vi "Scan Engine EtherCAT Generic Slave.vi"(8 "error in (no error)":errorcluster, 11 "Node Ptr":T1 format="%.0x") -> (0 "error out":errorcluster)   [LabVIEW 2027, in "SEECD System Explorer.lvlib"]
uses:
  SEECD System Explorer.lvlib
  <vilib>/NI VeriStand/Custom Device API/Custom Device Item Ref.ctl
  Shared/Globals/Property Strings.vi
  <vilib>/NI VeriStand/Custom Device API/Set Item Property (U16).vi
  <vilib>/NI VeriStand/Custom Device API/Set Item Property (Boolean).vi
  <vilib>/NI VeriStand/Custom Device API/Custom Device API.lvlib
  Shared/SEECD Shared.lvlib
  C:/NetCoreDLL/NationalInstruments.VeriStand.SystemDefinitionAPI.dll
  NetCoreDLL/NationalInstruments.VeriStand.SystemDefinitionAPI.dll
panel:
  in  "Enable Distributed Clock":bool caption="Enable distributed clock"
  out "ToString":string
  in  "Export to XML":bool
  in  "Prepend":bool caption="Prepend slave position to name"
  in  "SHDocVw.IWebBrowser2":refnum<k7>(container)
  in  "Slave Position":u16
  in  "Header":cluster{"Section Name":string}={"Section Name"="EtherCAT Slave"}
  in  "Name":string
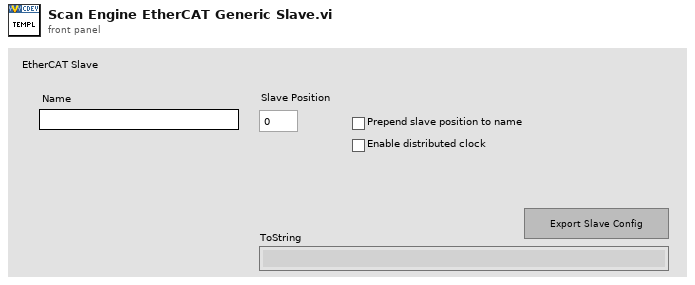
[diagram p1: front panel]
types:
  T1 = typedef "Custom Device API.lvlib/Custom Device Item Ref.ctl" = u64
  T2 = typedef "Custom Device API.lvlib/Custom Device Commands.ctl" = enum16{"Default", "Item renamed", "Shutdown", "Dynamic button pressed"}
  T3 = typedef "Custom Device API.lvlib/Custom Device Pointer.ctl" = refnum<k39>
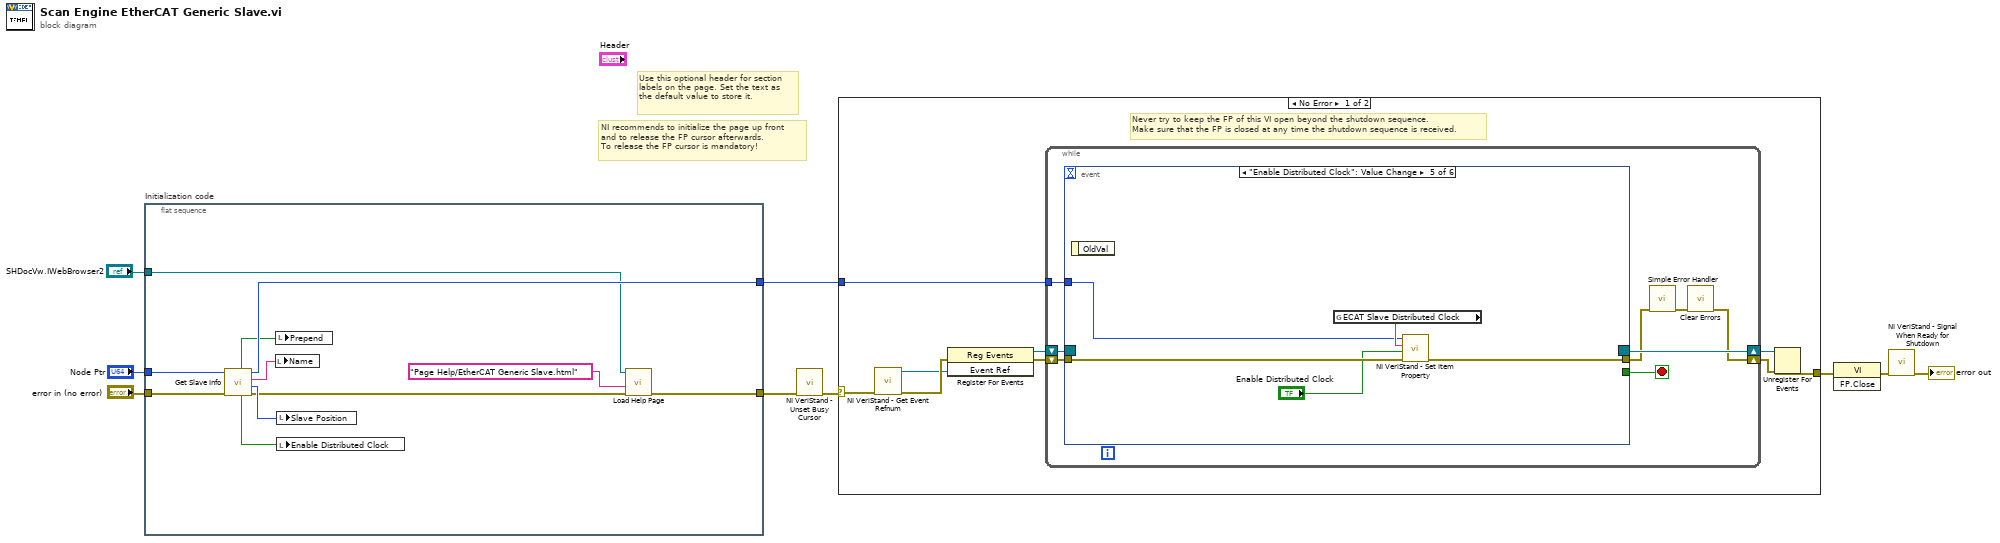
[diagram p0: block diagram]
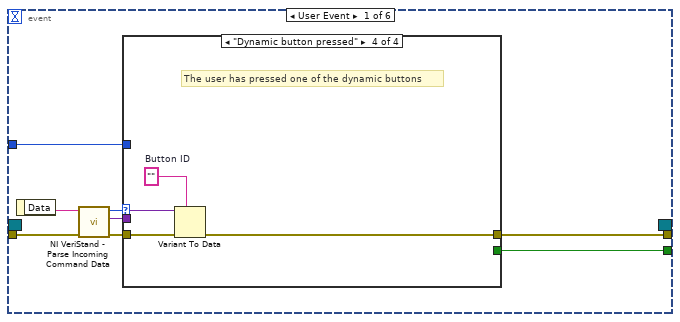
[diagram p2: hidden frame]
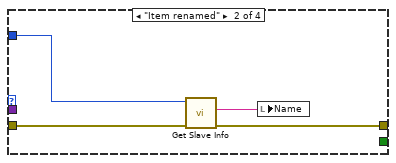
[diagram p4: hidden frame]
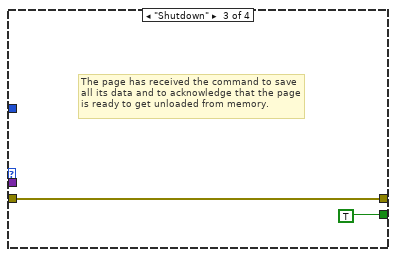
[diagram p5: hidden frame]
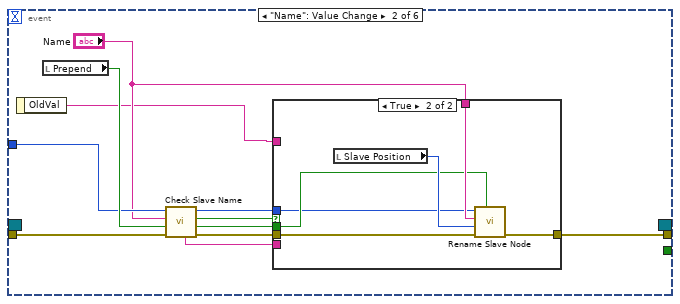
[diagram p6: hidden frame]
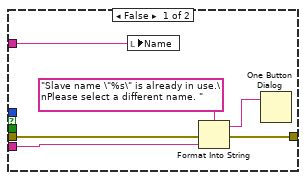
[diagram p7: hidden frame]
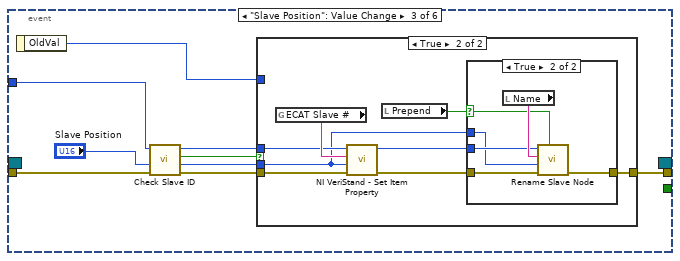
[diagram p8: hidden frame]
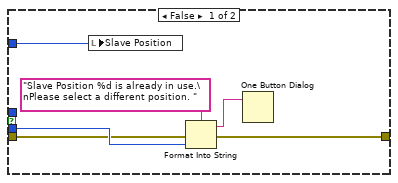
[diagram p9: hidden frame]
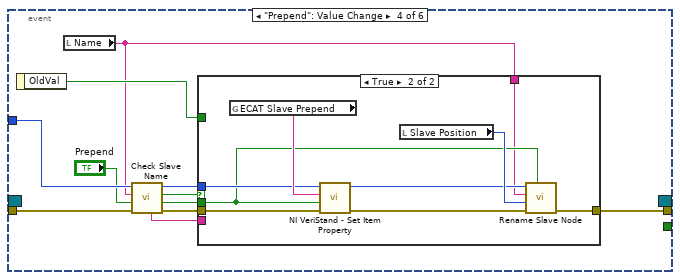
[diagram p11: hidden frame]
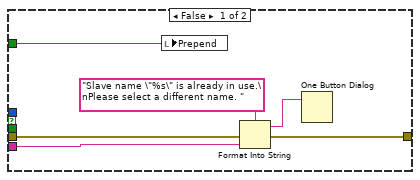
[diagram p12: hidden frame]
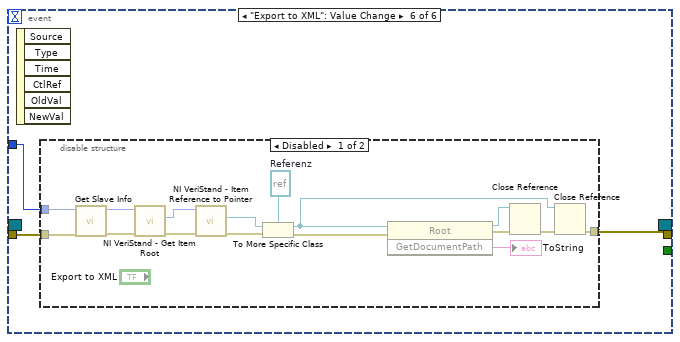
[diagram p13: hidden frame]
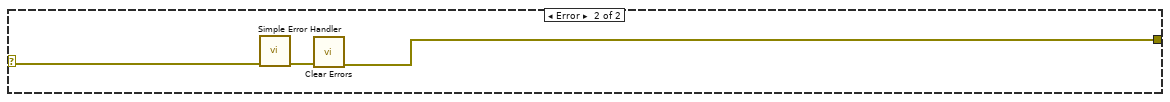
[diagram p15: hidden frame]
diagram:
  # "Use this optional header for section labels on the page. Set the text as the default value to store it."
  # "NI recommends to initialize the page up front\nand to release the FP cursor afterwards.\nTo release the FP cursor is mandatory!"
  n1 = flat-sequence "Initialization code" {
    tunnel: "error in (no error)" -> [w16]
    tunnel: "Node Ptr" -> [w17]
    tunnel: [w18] -> w3
    tunnel: "SHDocVw.IWebBrowser2" -> [w11]
    tunnel: [w12] -> w1
    frame #0 {
      n2 = call "Get Slave Info.vi"("error in (no error)"=w16, "Item Ref in"=w17) -> ("error out"=w13:errorcluster, "Slave #"=w19:u16, "Slave Name"=w20:string, "Item Ref out"=w18:T1, "Distributed Clock"=w10:bool, "Prepend"=w15:bool)  [unwired: 4 in]
      n3 = local write "Name"(w20) -> ()
      n4 = local write "Prepend"(w15) -> ()
      n5 = local write "Slave Position"(w19) -> ()
      n6 = local write "Enable Distributed Clock"(w10) -> ()
      n7 = call "Load Help Page.vi"("error in (no error)"=w13, "HTML File to Load"="Page Help/EtherCAT Generic Slave.html" ("name or relative path"), "Browser"=w11) -> ("error out"=w12:errorcluster)  [unwired: 8 in]
    }
  }
  n8 = call <vilib>:"NI VeriStand - Unset Busy Cursor.vi"("error in (no error)"=w1) -> ("error out"=w5:errorcluster)  [unwired: 10 out]
  n9 = case shown="No Error" w5 {
    selector: w5 -> [w21 w162]
    tunnel: [w26 w160] -> w9
    tunnel: w3 -> [w22 _]
    frame No Error {
      # "Never try to keep the FP of this VI open beyond the shutdown sequence.\nMake sure that the FP is closed at any time the shutdown sequence is received."
      n10 = call <vilib>:"NI VeriStand - Get Event Refnum.vi"("error in (no error)"=w21) -> ("error out"=w29:errorcluster, "Event Ref"=w25:refnum<user-event>)  [unwired: 9 out]
      n11 = register-events(error in=w29, w25) -> (reference out=w23:refnum<event-registration>, error out=w24:errorcluster)  [unwired: 1 in]
      n12 = while {
        tunnel: w22 -> [w33]
        shift-right: [w30] -> w27
        shift-left: w24 -> [w36]
        shift-right: [w37] -> w28
        shift-left: w23 -> [w35]
        stop <- w34 stop-if-true
        n13 = event shown="[4] \"Enable Distributed Clock\": Value Change" {
          selector: w35 -> [_ _ _ _ _ _]
          dyn-events: [_ _ _ _ _ _] -> w37
          timeout: _ -> [_ _ _ _ _ _]
          tunnel: w36 -> [w45 w60 w82 w118 w139 w143]
          tunnel: [w41 _ _ _ _ _] -> w34
          tunnel: [w40 w59 w80 w119 w138 w141] -> w32
          tunnel: w33 -> [w39 w61 w84 w117 w137 w142]
          event User Event {
            n14 = event-data() -> ("Data"=w44:string)  [unwired: 1 out]
            n15 = call <vilib>:"NI VeriStand - Parse Incoming Command Data.vi"("error in (no error)"=w45, "Incoming data"=w44) -> ("error out"=w43:errorcluster, "Outgoing data"=w38:variant, "Action"=w42:T2)  [unwired: 7 out]
            n16 = case shown="\"Dynamic button pressed\"" w42 {
              tunnel: w43 -> [w46 w50 w51 w56]
              tunnel: [_ _ TRUE _] -> w41
              tunnel: [w46 w49 w51 w53] -> w40
              tunnel: w39 -> [_ w47 _ _]
              tunnel: w38 -> [_ _ _ w55]
              frame "Default", Default {
              }
              frame "Item renamed" {
                n17 = call "Get Slave Info.vi"("error in (no error)"=w50, "Item Ref in"=w47) -> ("error out"=w49:errorcluster, "Slave Name"=w48:string)  [unwired: 4 in, 4 out]
                n18 = local write "Name"(w48) -> ()
              }
              frame "Shutdown" {
                # "The page has received the command to save all its data and to acknowledge that the page is ready to get unloaded from memory."
              }
              frame "Dynamic button pressed" {
                w54 = ""  # Button ID
                # "The user has pressed one of the dynamic buttons"
                n19 = Variant To Data(error in=w56, type=w54, Variant=w55) -> (error out=w53:errorcluster)  [unwired: 1 out]
              }
            }
          }
          event "Name": Value Change {
            n20 = event-data() -> ("OldVal"=w57:string)  [unwired: 1 out]
            n21 = local read "Prepend"() -> (w62:bool)
            n22 = call "Check Slave Name.vi"("error in (no error)"=w60, "Prepend in"=w62, "Slave Name In"="Name", "Item Ref in"=w61) -> ("error out"=w65:errorcluster, "Prepend out"=w64:bool, "Available?"=w66:bool, "Item Ref out"=w67:T1, "Slave Name"=w63:string)  [unwired: 3 in]
            n23 = case shown="True" w66 {
              tunnel: [w71 w79] -> w59
              tunnel: w65 -> [w72 w76]
              tunnel: w67 -> [_ w74]
              tunnel: w64 -> [_ w75]
              tunnel: w63 -> [w69 _]
              tunnel: "Name" -> [_ w77]
              tunnel: w57 -> [w68 _]
              frame False {
                n24 = local write "Name"(w68) -> ()
                n25 = Format Into String(format string="Slave name \"%s\" is already in use.\nPlease select a different name. ", error in=w72, w69) -> (resulting string=w70:string, error out=w71:errorcluster)  [unwired: 1 in]
                n26 = One Button Dialog(message=w70) -> ()  [unwired: 1 in, 1 out]
              }
              frame True {
                n27 = local read "Slave Position"() -> (w78:u16)
                n28 = call "Rename Slave Node.vi"("Prepend"=w75, "error in (no error)"=w76, "Slave #"=w78, "Slave Name"=w77, "Item Ref in"=w74) -> ("error out"=w79:errorcluster)  [unwired: 5 in, 1 out]
              }
            }
          }
          event "Slave Position": Value Change {
            n29 = event-data() -> ("OldVal"=w81:u16)  [unwired: 1 out]
            n30 = call "Check Slave ID.vi"("error in (no error)"=w82, "Slave ID in"="Slave Position", "Item Ref in"=w84) -> ("error out"=w88:errorcluster, "Slave ID out"=w86:u16, "Available?"=w87:bool, "Item Ref out"=w85:T1)  [unwired: 5 in]
            n31 = case shown="True" w87 {
              tunnel: [w90 w102] -> w80
              tunnel: w88 -> [w91 w100]
              tunnel: w85 -> [_ w98]
              tunnel: w86 -> [w93 w96]
              tunnel: w81 -> [w89 _]
              frame False {
                n32 = local write "Slave Position"(w89) -> ()
                n33 = Format Into String(format string="Slave Position %d is already in use.\nPlease select a different position. ", error in=w91, w93) -> (resulting string=w92:string, error out=w90:errorcluster)  [unwired: 1 in]
                n34 = One Button Dialog(message=w92) -> ()  [unwired: 1 in, 1 out]
              }
              frame True {
                n35 = global read "Property Strings.vi" "ECAT Slave #"() -> (w101:string)
                n36 = call-poly <vilib>:"NI VeriStand - Set Item Property.vi"("error in (no error)"=w100, "Value"=w96, "Property Name"=w101, "Item Ref in"=w98) -> ("error out"=w99:errorcluster, "Item Ref out"=w97:T1)  [unwired: 5 in, 1 out]
                n37 = local read "Prepend"() -> (w95:bool)
                n38 = case shown="True" w95 {
                  selector: w95 -> [_ w104]
                  tunnel: [w103 w109] -> w102
                  tunnel: w99 -> [w103 w107]
                  tunnel: w97 -> [_ w106]
                  tunnel: w96 -> [_ w105]
                  frame False {
                  }
                  frame True {
                    n39 = local read "Name"() -> (w108:string)
                    n40 = call "Rename Slave Node.vi"("Prepend"=w104, "error in (no error)"=w107, "Slave #"=w105, "Slave Name"=w108, "Item Ref in"=w106) -> ("error out"=w109:errorcluster)  [unwired: 5 in, 1 out]
                  }
                }
              }
            }
          }
          event "Prepend": Value Change {
            n41 = event-data() -> ("OldVal"=w120:bool)  [unwired: 1 out]
            n42 = local read "Name"() -> (w110:string)
            n43 = call "Check Slave Name.vi"("error in (no error)"=w118, "Prepend in"="Prepend", "Slave Name In"=w110, "Item Ref in"=w117) -> ("error out"=w113:errorcluster, "Prepend out"=w112:bool, "Available?"=w114:bool, "Item Ref out"=w115:T1, "Slave Name"=w111:string)  [unwired: 3 in]
            n44 = case shown="True" w114 {
              tunnel: [w123 w135] -> w119
              tunnel: w113 -> [w124 w132]
              tunnel: w115 -> [_ w130]
              tunnel: w112 -> [_ w128]
              tunnel: w120 -> [w126 _]
              tunnel: w111 -> [w121 _]
              tunnel: w110 -> [_ w127]
              frame False {
                n45 = local write "Prepend"(w126) -> ()
                n46 = Format Into String(format string="Slave name \"%s\" is already in use.\nPlease select a different name. ", error in=w124, w121) -> (resulting string=w122:string, error out=w123:errorcluster)  [unwired: 1 in]
                n47 = One Button Dialog(message=w122) -> ()  [unwired: 1 in, 1 out]
              }
              frame True {
                n48 = global read "Property Strings.vi" "ECAT Slave Prepend"() -> (w133:string)
                n49 = call-poly <vilib>:"NI VeriStand - Set Item Property.vi"("error in (no error)"=w132, "Value"=w128, "Property Name"=w133, "Item Ref in"=w130) -> ("error out"=w131:errorcluster, "Item Ref out"=w129:T1)  [unwired: 5 in, 1 out]
                n50 = local read "Slave Position"() -> (w134:u16)
                n51 = call "Rename Slave Node.vi"("Prepend"=w128, "error in (no error)"=w131, "Slave #"=w134, "Slave Name"=w127, "Item Ref in"=w129) -> ("error out"=w135:errorcluster)  [unwired: 5 in, 1 out]
              }
            }
          }
          event "Enable Distributed Clock": Value Change {
            n52 = event-data() -> ()  [unwired: 2 out]
            n53 = global read "Property Strings.vi" "ECAT Slave Distributed Clock"() -> (w140:string)
            n54 = call-poly <vilib>:"NI VeriStand - Set Item Property.vi"("error in (no error)"=w139, "Value"="Enable Distributed Clock", "Property Name"=w140, "Item Ref in"=w137) -> ("error out"=w138:errorcluster)  [unwired: 5 in, 2 out]
          }
          event "Export to XML": Value Change {
            n55 = event-data() -> ()  [unwired: 7 out]
            n56 = disable-structure shown="Disabled" {
              disable-tunnel: w143 -> [w159 _]
              disable-tunnel: w142 -> [w158 _]
              disable-tunnel: [w153 _] -> w141
              frame Disabled {
                w147 = refnum<k39> refnum  # Referenz
                n57 = call "Get Slave Info.vi"("error in (no error)"=w159, "Item Ref in"=w158) -> ("error out"=w157:errorcluster, "Item Ref out"=w149:T1)  [unwired: 4 in, 4 out]
                n58 = call <vilib>:"NI VeriStand - Get Item Root.vi"("error in (no error)"=w157, "Item Ref in"=w149) -> ("error out"=w150:errorcluster, "Root Ref out"=w146:T1)  [unwired: 6 in, 2 out]
                n59 = call <vilib>:"NI VeriStand - Item Reference to Pointer.vi"("error in (no error)"=w150, "Item Ref in"=w146) -> ("error out"=w152:errorcluster, "Node Pointer"=w145:T3)  [unwired: 6 in, 2 out]
                n60 = To More Specific Class(target class=w147, reference=w145, error in=w152) -> (specific class reference=w148:refnum<k39>, error out=w151:errorcluster)
                n61 = invoke class="Root" method="GetDocumentPath"(reference=w148, error in=w151) -> (reference out=w155:refnum<k39>, error out=w156:errorcluster, "GetDocumentPath"=→"ToString":string)  [unwired: 1 in]
                n62 = Close Reference(reference=w155, error in (no error)=w156) -> (error out=w154:errorcluster)
                n63 = Close Reference(reference=w148, error in (no error)=w154) -> (error out=w153:errorcluster)
              }
              frame Enabled {
              }
            }
          }
        }
        n64 = call <vilib>:"Simple Error Handler.vi"("error in (no error)"=w32) -> ("error out"=w31:errorcluster)  [unwired: 1 in, 7 out]
        n65 = call <vilib>:"Clear Errors.vi"("error in (no error)"=w31) -> ("error out"=w30:errorcluster)  [unwired: 1 in, 5 out]
      }
      n66 = Unregister For Events(event registration refnum=w28, error in=w27) -> (error out=w26:errorcluster)
    }
    frame Error {
      n67 = call <vilib>:"Simple Error Handler.vi"("error in (no error)"=w162) -> ("error out"=w161:errorcluster)  [unwired: 1 in, 7 out]
      n68 = call <vilib>:"Clear Errors.vi"("error in (no error)"=w161) -> ("error out"=w160:errorcluster)  [unwired: 1 in, 5 out]
    }
  }
  n69 = invoke class="VI" method="FP.Close"(error in=w9) -> (error out=w8:errorcluster)  [unwired: 2 in, 2 out]
  n70 = call <vilib>:"NI VeriStand - Signal When Ready for Shutdown.vi"("error in (no error)"=w8) -> ("error out"=→"error out":errorcluster)  [unwired: 10 out]
